vi "QueryIR.vi"() -> (2 "Tick Count":u32, 3 "Is there an object?":bool)   [LabVIEW 2026]
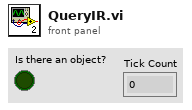
[diagram p1: front panel]
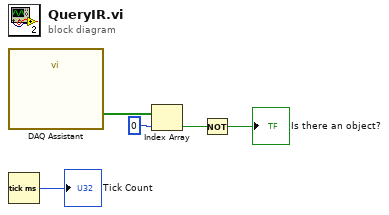
[diagram p0: block diagram]
diagram:
  n1 = call "DAQ Assistant"() -> ("data"=w4:bool[])  [unwired: 17 in, 2 out]
  n2 = Tick Count (ms)() -> (millisecond timer value=→"Tick Count":u32)
  n3 = Index Array(array=w4, index=0) -> (element=w5:bool)
  n4 = Not(x=w5) -> (.not. x?=→"Is there an object?":bool)
